vi "midiInOpen.vi"(7 "Event Filter":u8[](array[numeric])=[128, 144, 176] format="%.0x", 8 "error in":errorcluster, 9 "midi-callback-userevent":refnum<class "midi-callback-userevent.lvclass">, 10 "MIDI Device ID":u32, 11 "midi in":refnum<class "midi.lvclass">) -> (0 "error out":errorcluster, 3 "midi out":refnum<class "midi.lvclass">)   [LabVIEW 2020, in "midi.lvclass"]
doc: "The midiInOpen function opens a specified MIDI input device."
uses:
  midi.lvclass
  midi.lvclass/midi.ctl
  cpp-src/MIDIInToLabVIEWWrapper/x64/Release/MIDIInToLabVIEWWrapper.dll
  midi-callback-userevent/midi-callback-userevent.lvclass
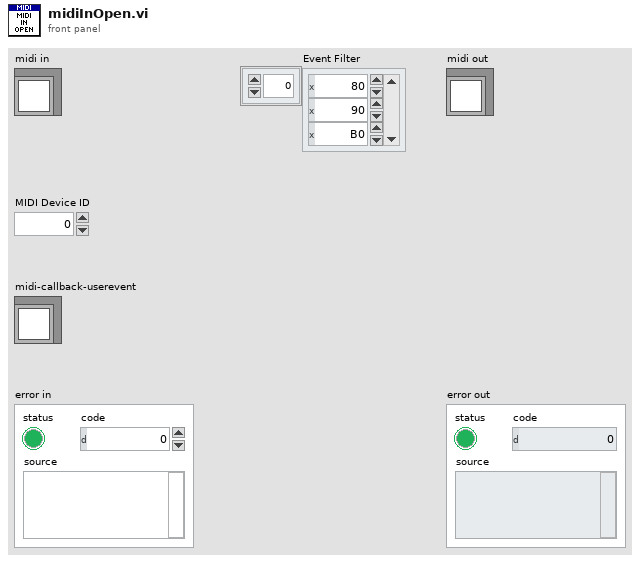
[diagram p1: front panel]
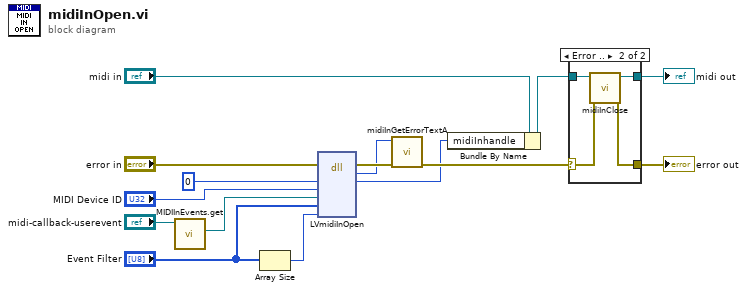
[diagram p0: block diagram]
diagram:
  n1 = call "MIDIInEvents.get.vi"("midi-callback-userevent"="midi-callback-userevent") -> ("MIDIInEvents"=w3:refnum<user-event>)  [unwired: 10 in]
  n2 = Array Size(array="Event Filter") -> (size(s)=w7:i32)
  n3 = dll-call lib="C:/code/LabVIEW-MIDI/cpp-src/MIDIInToLabVIEWWrapper/x64/Release/MIDIInToLabVIEWWrapper.dll" fn="LVmidiInOpen"(error in="error in", "phMidiIn"=u64 0 ("hMidiIn"), "uDeviceID"="MIDI Device ID", "pUserEventRef"=w3, "filterArray"="Event Filter", "arraySize"=w7) -> (error out=w5:errorcluster, "error"=w2:i32, "phMidiIn"=w1:u64)  [unwired: 6 in, 1 out]
  n4 = call "midiInGetErrorTextA.vi"("error in"=w5, "Error Code"=w2) -> ("error out"=w9:errorcluster)  [unwired: 9 in]
  n5 = Bundle By Name(cluster="midi in", "midiInhandle"=w1) -> (w14:refnum<class "midi.lvclass">)
  n6 = case shown="Error .." w9 {
    selector: w9 -> [w16 w18]
    tunnel: w14 -> [w17 w21]
    tunnel: [w17 w20] -> w13
    tunnel: [w16 w19] -> w12
    frame No Error {
    }
    frame Error {
      n7 = call "midiInClose.vi"("error in"=w18, "midi in"=w21) -> ("error out"=w19:errorcluster, "midi out"=w20:refnum<class "midi.lvclass">)  [unwired: 8 in]
    }
  }
  "midi out" <- w13
  "error out" <- w12
